vi "Registry Test Launcher.vi"() -> ()   [LabVIEW 2013]
uses:
  UniquenessCriteria/Criteria.ctl
  StringIncrement/StringIncrement.lvclass
  StringIncrement.Alphabetical/StringIncrement.Alphabetical.lvclass
  UniqueNameClass/UniqueName.lvclass/UniqueName.ctl
  Registry/NameRegistry.lvclass
  UniquenessCriteria/UniquenessCriteria.lvclass
  UniqueNameClass/UniqueName.lvclass
panel:
  in  "Increment Function":enum16{"Numerical", "Alphabetical"}(ring)
  in  "Criteria":T1
  out "All Nodes":string[](array[string])
  out "objects remaining":i32
  out "error out":errorcluster
  out "Dependencies removed":string[](array[string])
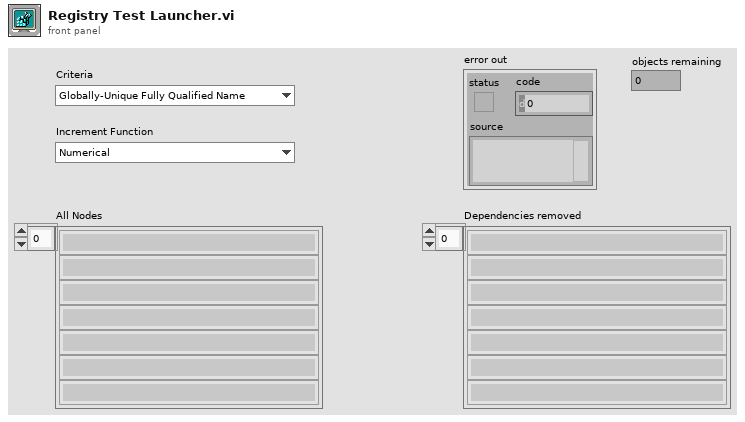
[diagram p1: front panel]
types:
  T1 = typedef "UniqueName.lvlib/UniquenessCriteria.lvclass/Criteria.ctl" = enum16{"Globally-Unique Fully Qualified Name", "Globally-Unique Name", "Universal Unique Identifier"}
  T2 = typedef "UniqueName.lvlib/NameRegistry.lvclass/RegistryConfiguration.ctl" = cluster{"Delimiter":refnum<class "Delimiter.lvclass">, "RandomStringGenerator":refnum<class "RandomStringGenerator.lvclass">, "UniquenessCriteria":refnum<class "UniquenessCriteria.lvclass">, "StringIncrement":refnum<class "StringIncrement.lvclass">}
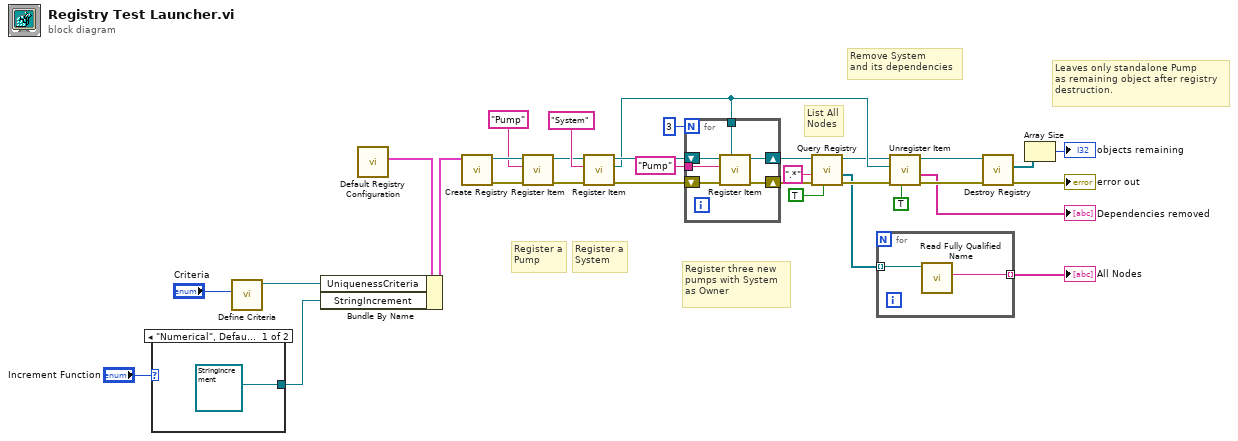
[diagram p0: block diagram]
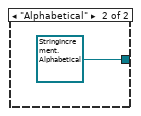
[diagram p2: hidden frame]
diagram:
  # "Leaves only standalone Pump\nas remaining object after registry\ndestruction."
  # "Remove System\nand its dependencies"
  # "List All\nNodes"
  # "Register three new\npumps with System\nas Owner"
  # "Register a\nSystem"
  # "Register a\nPump"
  n1 = case shown="\"Numerical\", Default" "Increment Function" {
    tunnel: [refnum<class "StringIncrement.lvclass"> refnum ("StringIncrement.lvclass") refnum<class "StringIncrement.Alphabetical.lvclass"> refnum ("StringIncrement.Alphabetical.lvclass")] -> w2
    frame "Numerical", Default {
    }
    frame "Alphabetical" {
    }
  }
  n2 = call "Define Criteria.vi"("Criteria"="Criteria") -> ("UniquenessCriteria out"=w18:refnum<class "UniquenessCriteria.lvclass">)  [unwired: 10 in]
  n3 = call "Default Registry Configuration.vi"() -> ("Registry Configuration"=w1:T2)  [unwired: 11 in]
  n4 = Bundle By Name(cluster=w1, "UniquenessCriteria"=w18, "StringIncrement"=w2) -> (w19:T2)
  n5 = call "Create Registry.vi"("Registry Configuration"=w19) -> ("error out"=w14:errorcluster, "Registry"=w15:refnum<data-value>)  [unwired: 9 in]
  n6 = call "Register Item.vi"("error in (no error)"=w14, "New Object Name"="Pump", "Registry in"=w15) -> ("error out"=w16:errorcluster, "Registry"=w17:refnum<data-value>)  [unwired: 6 in, 1 out]
  n7 = call "Register Item.vi"("error in (no error)"=w16, "New Object Name"="System", "Registry in"=w17) -> ("error out"=w30:errorcluster, "New Node"=w21:refnum<class "UniqueName.lvclass">, "Registry"=w31:refnum<data-value>)  [unwired: 6 in]
  n8 = for {
    N: 3 -> [_]
    shift-right: [w39] -> w12
    shift-left: w31 -> [w40]
    shift-right: [w37] -> w10
    shift-left: w30 -> [w38]
    tunnel: "Pump" ("New Object Name") -> [w36]
    tunnel: w21 -> [w35]
    n9 = call "Register Item.vi"("Owner"=w35, "error in (no error)"=w38, "New Object Name"=w36, "Registry in"=w40) -> ("error out"=w37:errorcluster, "Registry"=w39:refnum<data-value>)  [unwired: 5 in, 1 out]
  }
  n10 = call "Query Registry.vi"("use Regex? (F)"=TRUE, "error in (no error)"=w10, "Search string"=".*", "Registry in"=w12) -> ("error out"=w9:errorcluster, "Nodes"=w6:refnum<class "UniqueName.lvclass">[], "Registry"=w11:refnum<data-value>)  [unwired: 3 in, 2 out]
  n11 = for {
    tunnel: w6 -> [w42] mode=indexing
    tunnel: [w41] -> w5 mode=indexing
    n12 = call "Read Fully Qualified Name.vi"("UniqueName in"=w42) -> ("Fully Qualified Name"=w41:string)  [unwired: 9 in, 1 out]
  }
  "All Nodes" <- w5
  n13 = call "Unregister Item.vi"("Remove Dependencies?"=TRUE, "error in (no error)"=w9, "Node"=w21, "Registry in"=w11) -> ("error out"=w28:errorcluster, "Dependencies removed"=→"Dependencies removed":string[], "Registry"=w32:refnum<data-value>)  [unwired: 4 in, 1 out]
  n14 = call "Destroy Registry.vi"("error in (no error)"=w28, "Registry in"=w32) -> ("error out"=→"error out":errorcluster, "Remaining Nodes"=w4:refnum<class "UniqueName.lvclass">[])  [unwired: 8 in]
  n15 = Array Size(array=w4) -> (size(s)=→"objects remaining":i32)
